vi "DT-Calibration.vi"(8 "error in":errorcluster, 11 "Calibration in":refnum<class "Calibration.lvclass">) -> (0 "error out":errorcluster, 3 "Calibration out":refnum<class "Calibration.lvclass">)   [LabVIEW 2022 SP3, in "Bontech Calibration.lvlib" / "Calibration.lvclass"]
uses:
  Calibration.lvclass
  Calibration.lvclass/Calibration.ctl
  xPanelWrapperLvLib/xPanelWrapper.lvlib
  d077555a-1f94-446a-85b2-7b0ad1c6b4f0.vi
  db90e855-191f-4739-9521-1b2d8c1b96f4.vi
  10b23209-33a3-4e9b-93f0-ebaa28cb70a6.vi
panel:
  out "DefectValid?":bool
  in  "Defect":bool
  in  "No of Frames for Calibration (10 - 50)":u16=20 min=100 max=10000
  out "GainValid?":bool
  out "OffsetValid?":bool
  in  "Status":string
  in  "Gain":bool
  in  "Offset":bool
  # "Aayvu  Calibration Tool"
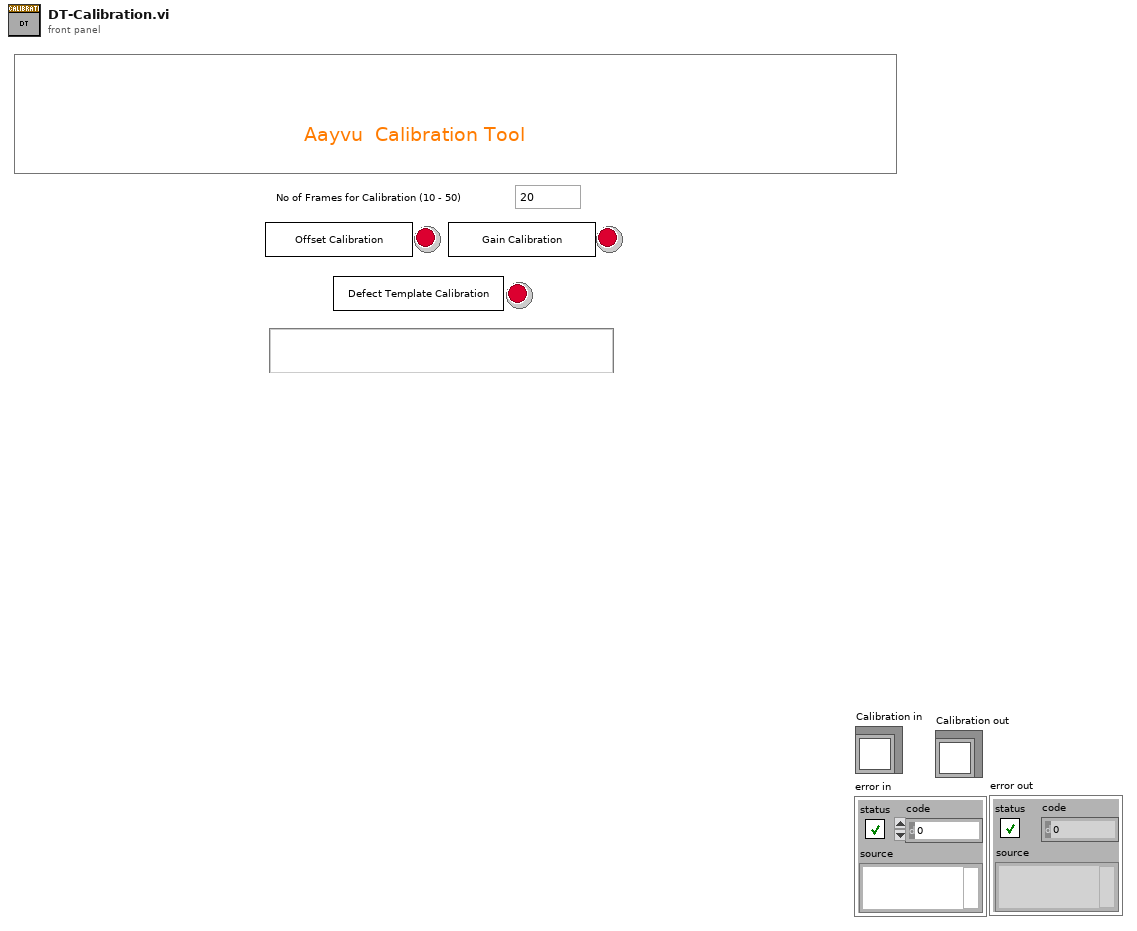
[diagram p1: front panel]
types:
  T1 = typedef "Paths.ctl" = cluster{"Configuration":path, "Event Logs":path, "Error Logs":path, "Calibration":path, "Settings.ini":path, "UserInfo.bin":path, "TimeStamp File":path, "FileCounter.txt":path}
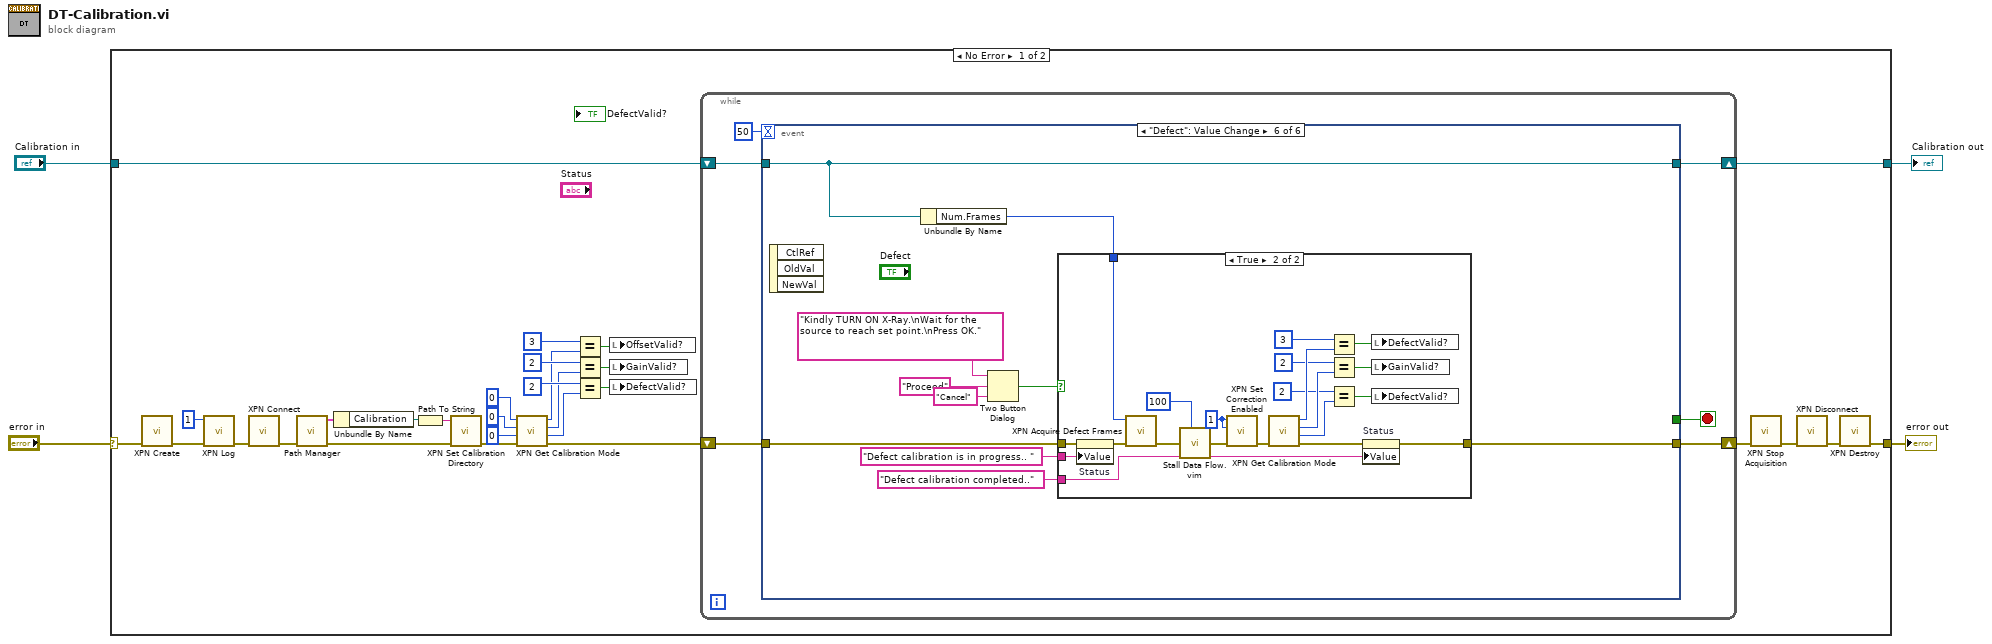
[diagram p0: block diagram]
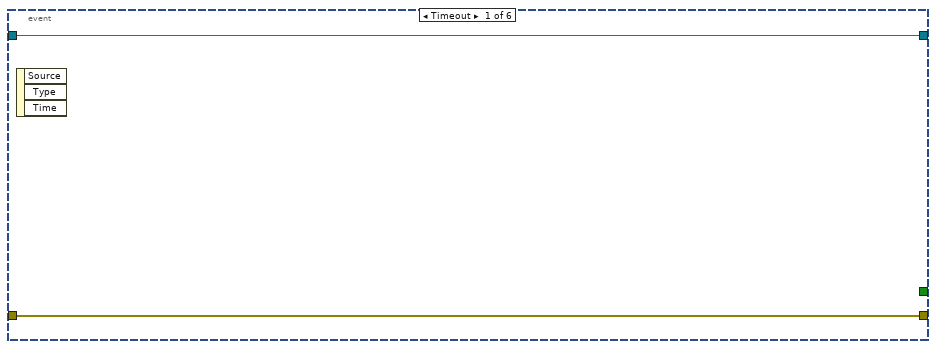
[diagram p2: hidden frame]
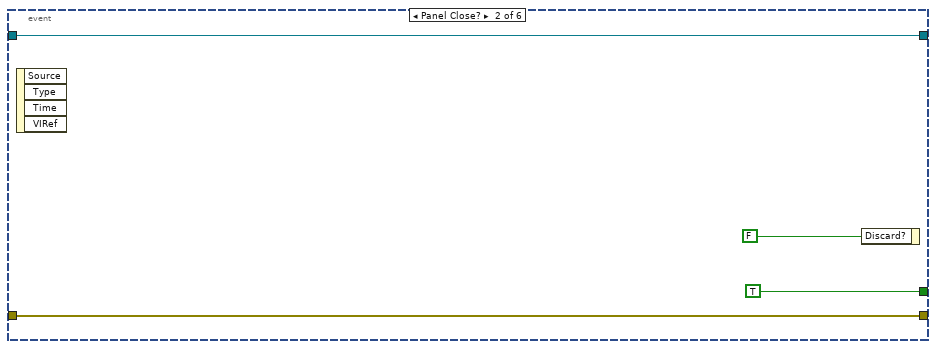
[diagram p3: hidden frame]
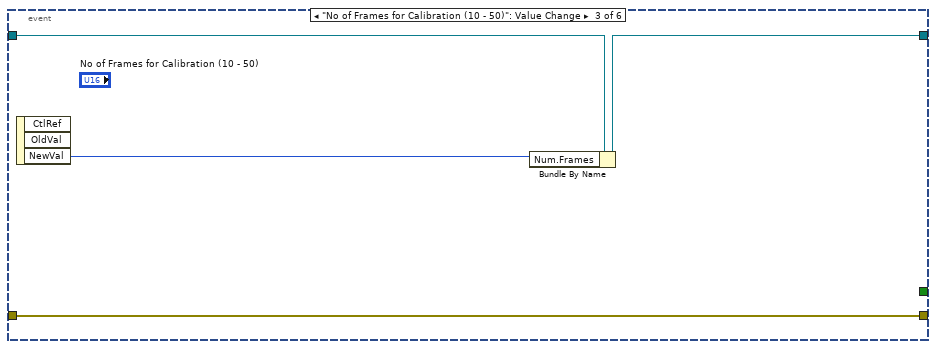
[diagram p4: hidden frame]
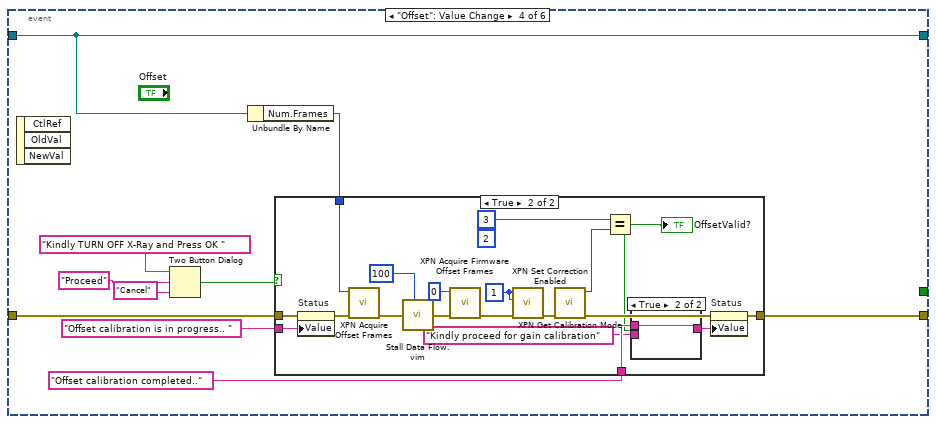
[diagram p5: hidden frame]
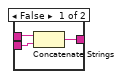
[diagram p7: hidden frame]
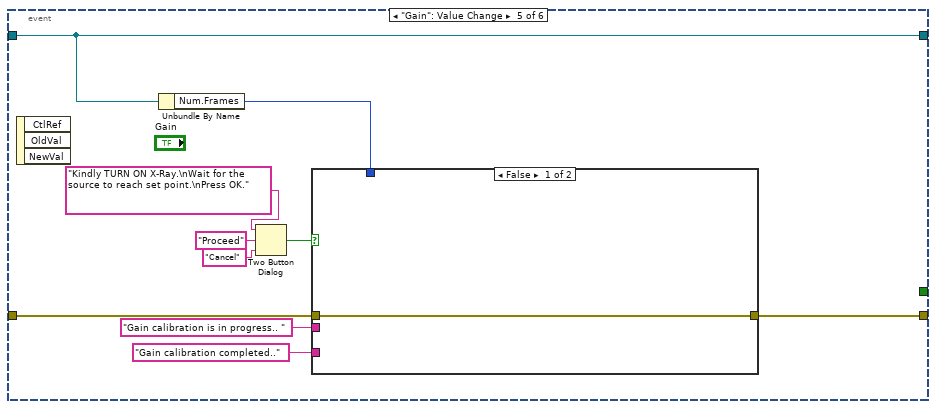
[diagram p8: hidden frame]
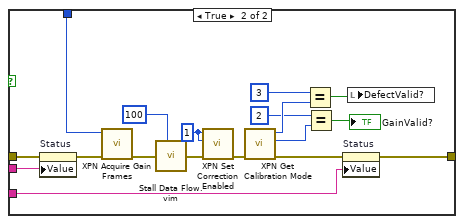
[diagram p9: hidden frame]
diagram:
  n1 = case shown="No Error" "error in" {
    selector: "error in" -> [w31 w146]
    tunnel: [w14 w146] -> w3
    tunnel: [w32 w145] -> w1
    tunnel: "Calibration in" -> [w33 w145]
    frame No Error {
      n2 = call "XPN Create.vi"("error in (no error)"=w31) -> ("error out"=w13:errorcluster)  [unwired: 9 in, 1 out]
      n3 = call "XPN Log.vi"("error in (no error)"=w13, "enable"=1) -> ("error out"=w12:errorcluster)  [unwired: 8 in, 1 out]
      n4 = call "XPN Connect.vi"("error in (no error)"=w12) -> ("error out"=w10:errorcluster)  [unwired: 9 in, 1 out]
      n5 = call "Path Manager.vi"("error in (no error)"=w10) -> ("Cluster"=w7:T1, "Error out"=w8:errorcluster)  [unwired: 13 in]
      n6 = Unbundle By Name(w7) -> ("Calibration"=w6:path)
      n7 = Path To String(path=w6) -> (string=w5:string)
      n8 = call "XPN Set Calibration Directory.vi"("error in (no error)"=w8, "dirPath"=w5) -> ("error out"=w9:errorcluster)  [unwired: 8 in, 1 out]
      n9 = call "XPN Get Calibration Mode.vi"("error in (no error)"=w9, "defectMode"=0 ("numFrames"), "gainMode"=0 ("numFrames"), "offsetMode"=0 ("numFrames")) -> ("error out"=w29:errorcluster, "defectMode out"=w20:i32, "gainMode out"=w21:i32, "offsetMode out"=w22:i32)  [unwired: 3 in, 1 out]
      n10 = Equal?(x=3 ("numFrames"), y=w22) -> (x = y?=w19:bool)
      n11 = Equal?(x=2 ("numFrames"), y=w21) -> (x = y?=w18:bool)
      n12 = Equal?(x=2 ("numFrames"), y=w20) -> (x = y?=w17:bool)
      n13 = local write "OffsetValid?"(w19) -> ()
      n14 = local write "GainValid?"(w18) -> ()
      n15 = local write "DefectValid?"(w17) -> ()
      n16 = while {
        shift-right: [w38] -> w32
        shift-left: w33 -> [w39]
        shift-right: [w36] -> w30
        shift-left: w29 -> [w37]
        stop <- w34 stop-if-true
        n17 = event shown="[5] \"Defect\": Value Change" {
          selector: _ -> [_ _ _ _ _ _]
          dyn-events: _ -> [_ _ _ _ _ _]
          timeout: 50 -> [_ _ _ _ _ _]
          tunnel: w39 -> [w41 w45 w49 w58 w91 w120]
          tunnel: [w41 w45 w47 w58 w91 w120] -> w38
          tunnel: [w40 w44 w48 w56 w92 w121] -> w36
          tunnel: w37 -> [w40 w44 w48 w59 w93 w122]
          tunnel: [_ TRUE _ _ _ _] -> w34
          event Timeout {
            n18 = event-data() -> ()  [unwired: 1 in, 3 out]
          }
          event Panel Close? {
            n19 = event-data() -> ()  [unwired: 1 in, 4 out]
            n20 = event-data("Discard?"=FALSE) -> ()  [unwired: 1 in, 1 out]
          }
          event "No of Frames for Calibration (10 - 50)": Value Change {
            n21 = event-data() -> ("NewVal"=w46:u16)  [unwired: 1 in, 2 out]
            n22 = Bundle By Name(cluster=w49, "Num.Frames"=w46) -> (w47:refnum<class "Calibration.lvclass">)
          }
          event "Offset": Value Change {
            n23 = event-data() -> ()  [unwired: 1 in, 3 out]
            n24 = Two Button Dialog(message="Kindly TURN OFF X-Ray and Press OK " ("Value"), 1:"Cancel" ("F button name (\"Cancel\")"), 2:"Proceed" ("T button name (\"OK\")")) -> (T button?=w50:bool)
            n25 = Unbundle By Name(w58) -> ("Num.Frames"=w57:u16)
            n26 = case shown="True" w50 {
              tunnel: w59 -> [w60 w79]
              tunnel: w57 -> [_ w73]
              tunnel: [w60 w66] -> w56
              tunnel: "Offset calibration completed.." ("Value") -> [_ w65]
              tunnel: "Offset calibration is in progress.. " ("Value") -> [_ w61]
              frame False {
              }
              frame True {
                w68 = 1 ("numFrames")
                (unwired) 2 ("numFrames")
                n27 = property on="Status" class="Str"(error in=w79, "Value"=w61) -> (error out=w67:errorcluster)  [unwired: 1 in, 1 out]
                n28 = call "XPN Acquire Offset Frames.vi"("error in (no error)"=w67, "numFrames"=w73) -> ("error out"=w78:errorcluster)  [unwired: 8 in, 1 out]
                n29 = call "Stall Data Flow.vim"("value in"=w78, "milliseconds to wait"=u32 100) -> ("value out"=w77:errorcluster)  [unwired: 1 out]
                n30 = call "XPN Acquire Firmware Offset Frames.vi"("error in (no error)"=w77, "numFrames"=0) -> ("error out"=w76:errorcluster)  [unwired: 8 in, 1 out]
                n31 = call "XPN Set Correction Enabled.vi"("error in (no error)"=w76, "enableGain"=w68, "enableOffset"=w68) -> ("error out"=w75:errorcluster)  [unwired: 7 in, 1 out]
                n32 = call "XPN Get Calibration Mode.vi"("error in (no error)"=w75) -> ("error out"=w74:errorcluster, "offsetMode out"=w71:i32)  [unwired: 6 in, 3 out]
                n33 = Equal?(x=3 ("numFrames"), y=w71) -> (x = y?=w63:bool)
                "OffsetValid?" <- w63
                n34 = case shown="True" w63 {
                  tunnel: w65 -> [w82 w83]
                  tunnel: [w81 w83] -> w64
                  tunnel: "Kindly proceed for gain calibration" ("Value") -> [w80 _]
                  frame False {
                    n35 = Concatenate Strings(w82, w80) -> (w81:string)
                  }
                  frame True {
                  }
                }
                n36 = property on="Status" class="Str"(error in=w74, "Value"=w64) -> (error out=w66:errorcluster)  [unwired: 1 in, 1 out]
              }
            }
          }
          event "Gain": Value Change {
            n37 = event-data() -> ()  [unwired: 1 in, 3 out]
            n38 = Unbundle By Name(w91) -> ("Num.Frames"=w90:u16)
            n39 = Two Button Dialog(message="Kindly TURN ON X-Ray.\nWait for the source to reach set point.\nPress OK." ("Value"), 1:"Cancel" ("F button name (\"Cancel\")"), 2:"Proceed" ("T button name (\"OK\")")) -> (T button?=w87:bool)
            n40 = case shown="False" w87 {
              tunnel: w93 -> [w94 w112]
              tunnel: [w94 w97] -> w92
              tunnel: w90 -> [_ w107]
              tunnel: "Gain calibration is in progress.. " ("Value") -> [_ w96]
              tunnel: "Gain calibration completed.." ("Value") -> [_ w95]
              frame False {
              }
              frame True {
                w104 = 1 ("numFrames")
                n41 = property on="Status" class="Str"(error in=w112, "Value"=w96) -> (error out=w98:errorcluster)  [unwired: 1 in, 1 out]
                n42 = call "XPN Acquire Gain Frames.vi"("error in (no error)"=w98, "numFrames"=w107) -> ("error out"=w111:errorcluster)  [unwired: 8 in, 1 out]
                n43 = call "Stall Data Flow.vim"("value in"=w111, "milliseconds to wait"=u32 100) -> ("value out"=w110:errorcluster)  [unwired: 1 out]
                n44 = call "XPN Set Correction Enabled.vi"("error in (no error)"=w110, "enableGain"=w104, "enableOffset"=w104) -> ("error out"=w109:errorcluster)  [unwired: 7 in, 1 out]
                n45 = call "XPN Get Calibration Mode.vi"("error in (no error)"=w109) -> ("error out"=w108:errorcluster, "gainMode out"=w102:i32, "offsetMode out"=w106:i32)  [unwired: 6 in, 2 out]
                n46 = Equal?(x=3 ("numFrames"), y=w106) -> (x = y?=w99:bool)
                n47 = Equal?(x=2 ("numFrames"), y=w102) -> (x = y?=→"GainValid?":bool)
                n48 = property on="Status" class="Str"(error in=w108, "Value"=w95) -> (error out=w97:errorcluster)  [unwired: 1 in, 1 out]
                n49 = local write "DefectValid?"(w99) -> ()
              }
            }
          }
          event "Defect": Value Change {
            n50 = event-data() -> ()  [unwired: 1 in, 3 out]
            n51 = Unbundle By Name(w120) -> ("Num.Frames"=w119:u16)
            n52 = Two Button Dialog(message="Kindly TURN ON X-Ray.\nWait for the source to reach set point.\nPress OK." ("Value"), 1:"Cancel" ("F button name (\"Cancel\")"), 2:"Proceed" ("T button name (\"OK\")")) -> (T button?=w115:bool)
            n53 = case shown="True" w115 {
              tunnel: w122 -> [w123 w128]
              tunnel: [w123 w126] -> w121
              tunnel: w119 -> [_ w140]
              tunnel: "Defect calibration is in progress.. " ("Value") -> [_ w125]
              tunnel: "Defect calibration completed.." ("Value") -> [_ w124]
              frame False {
              }
              frame True {
                w137 = 1 ("numFrames")
                n54 = property on="Status" class="Str"(error in=w128, "Value"=w125) -> (error out=w127:errorcluster)  [unwired: 1 in, 1 out]
                n55 = call "XPN Acquire Defect Frames.vi"("error in (no error)"=w127, "numFrames"=w140) -> ("error out"=w144:errorcluster)  [unwired: 8 in, 1 out]
                n56 = call "Stall Data Flow.vim"("value in"=w144, "milliseconds to wait"=u32 100) -> ("value out"=w143:errorcluster)  [unwired: 1 out]
                n57 = call "XPN Set Correction Enabled.vi"("error in (no error)"=w143, "enableGain"=w137, "enableOffset"=w137) -> ("error out"=w142:errorcluster)  [unwired: 7 in, 1 out]
                n58 = call "XPN Get Calibration Mode.vi"("error in (no error)"=w142) -> ("error out"=w141:errorcluster, "defectMode out"=w130:i32, "gainMode out"=w135:i32, "offsetMode out"=w139:i32)  [unwired: 6 in, 1 out]
                n59 = Equal?(x=3 ("numFrames"), y=w139) -> (x = y?=w133:bool)
                n60 = Equal?(x=2 ("numFrames"), y=w135) -> (x = y?=w132:bool)
                n61 = Equal?(x=2 ("numFrames"), y=w130) -> (x = y?=w131:bool)
                n62 = property on="Status" class="Str"(error in=w141, "Value"=w124) -> (error out=w126:errorcluster)  [unwired: 1 in, 1 out]
                n63 = local write "DefectValid?"(w133) -> ()
                n64 = local write "GainValid?"(w132) -> ()
                n65 = local write "DefectValid?"(w131) -> ()
              }
            }
          }
        }
      }
      n66 = call "XPN Stop Acquisition.vi"("error in (no error)"=w30) -> ("error out"=w16:errorcluster)  [unwired: 9 in, 1 out]
      n67 = call "XPN Disconnect.vi"("error in (no error)"=w16) -> ("error out"=w15:errorcluster)  [unwired: 9 in, 1 out]
      n68 = call "XPN Destroy.vi"("error in (no error)"=w15) -> ("error out"=w14:errorcluster)  [unwired: 9 in, 1 out]
    }
    frame Error {
    }
  }
  "error out" <- w3
  "Calibration out" <- w1
